vi "subFindProjects.vi"(8 "error in (no error)":errorcluster, 11 "SolutionBuilder in":refnum<class "SolutionBuilder.lvclass">) -> (0 "error out":errorcluster, 3 "SolutionBuilder out":refnum<class "SolutionBuilder.lvclass">)   [LabVIEW 2019, in "SolutionBuilder.lvlib" / "SolutionBuilder.lvclass"]
uses:
  SolutionBuilder.lvclass
  SolutionBuilder.lvclass/SolutionBuilder.ctl
  ProjectItem/ProjectItem.lvclass
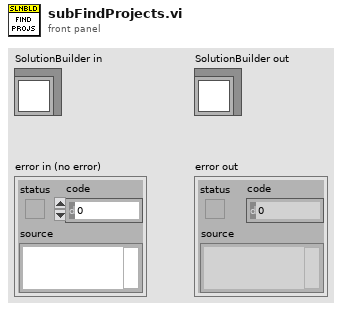
[diagram p1: front panel]
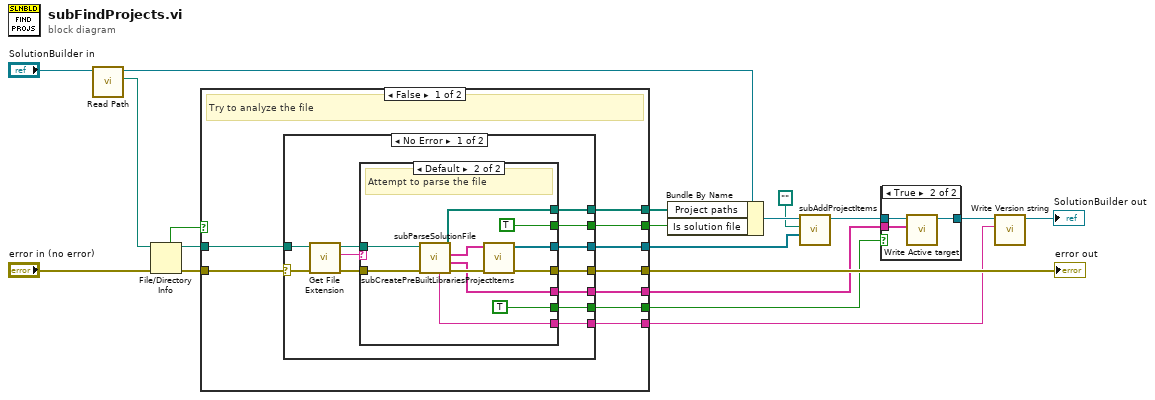
[diagram p0: block diagram]
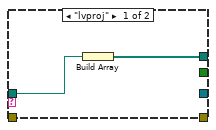
[diagram p3: hidden frame]
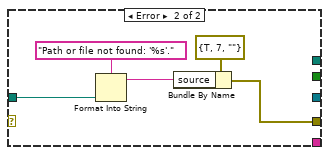
[diagram p4: hidden frame]
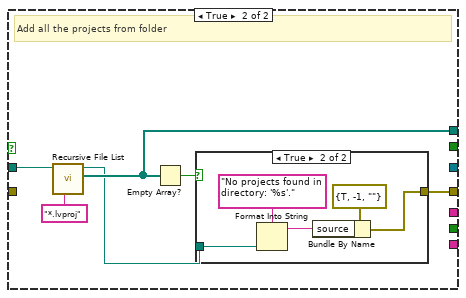
[diagram p5: hidden frame]
diagram:
  n1 = call "Read Path.vi"("SolutionBuilder in"="SolutionBuilder in") -> ("Path"=w15:path, "SolutionBuilder out"=w14:refnum<class "SolutionBuilder.lvclass">)  [unwired: 9 in]
  n2 = File/Directory Info(path=w15, error in="error in (no error)") -> (path out=w18:path, directory=w19:bool, error out=w17:errorcluster)  [unwired: 4 out]
  n3 = case shown="False" w19 {
    tunnel: [w26 w62] -> w11
    tunnel: w18 -> [w28 w61]
    tunnel: w17 -> [w27 _]
    tunnel: [w25 w63] -> w12
    tunnel: [w24 _] -> w8
    tunnel: [w23 _] -> w7
    tunnel: [w22 _] -> w5
    tunnel: [w21 _] -> w4
    tunnel: [w20 _] -> w1
    frame False {
      # "Try to analyze the file"
      n4 = case shown="No Error" w27 {
        selector: w27 -> [w39 _]
        tunnel: w28 -> [w38 w56]
        tunnel: [w40 _] -> w26
        tunnel: [w34 w55] -> w25
        tunnel: [w33 _] -> w24
        tunnel: [w32 _] -> w23
        tunnel: [w31 _] -> w22
        tunnel: [w30 _] -> w21
        tunnel: [w29 _] -> w20
        frame No Error {
          n5 = call <vilib>:"Get File Extension.vi"("error in (no error)"=w39, "file"=w38) -> ("error out"=w36:errorcluster, "lowercase file extension"=w35:string, "dup file"=w37:path)  [unwired: 5 in, 2 out]
          n6 = case shown="Default" w35 {
            tunnel: [w41 w53] -> w40
            tunnel: w37 -> [w42 w51]
            tunnel: w36 -> [_ w52]
            tunnel: [_ w48] -> w34
            tunnel: [_ w47] -> w33
            tunnel: [_ TRUE ("Is solution file")] -> w32
            tunnel: [_ w45] -> w31
            tunnel: [_ TRUE] -> w30
            tunnel: [_ w43] -> w29
            frame "lvproj" {
              n7 = Build Array(w42) -> (w41:path[])
            }
            frame Default {
              # "Attempt to parse the file"
              n8 = call "subParseSolutionFile.vi"("error in (no error)"=w52, "Solution file"=w51) -> ("error out"=w49:errorcluster, "Active targets"=w45:string[], "Lib definition strings"=w50:string[], "Projects"=w53:path[], "Version string"=w43:string)  [unwired: 5 in]
              n9 = call "subCreatePreBuiltLibrariesProjectItems.vi"("error in"=w49, "Lib definition strings"=w50) -> ("error out"=w48:errorcluster, "Pre-built libraries"=w47:refnum<class "ProjectItem.lvclass">[])  [unwired: 8 in]
            }
          }
        }
        frame Error {
          n10 = Format Into String(format string="Path or file not found: '%s'.", w56) -> (resulting string=w57:string)  [unwired: 2 in, 1 out]
          n11 = Bundle By Name(cluster=errorcluster {"status"=TRUE, "code"=7, "source"=""} ("t"), "source"=w57) -> (w55:errorcluster)
        }
      }
    }
    frame True {
      # "Add all the projects from folder"
      n12 = call <vilib>:"Recursive File List.vi"("pattern"="*.lvproj", "Folder Path"=w61) -> ("All Files in Dir"=w62:path[], "dup Folder Path"=w60:path)  [unwired: 5 in, 3 out]
      n13 = Empty Array?(array=w62) -> (empty?=w59:bool)
      n14 = case shown="True" w59 {
        tunnel: [_ w66] -> w63
        tunnel: w60 -> [_ w65]
        frame False {
        }
        frame True {
          n15 = Format Into String(format string="No projects found in directory: '%s'.", w65) -> (resulting string=w68:string)  [unwired: 2 in, 1 out]
          n16 = Bundle By Name(cluster=errorcluster {"status"=TRUE, "code"=-1, "source"=""} ("t"), "source"=w68) -> (w66:errorcluster)
        }
      }
    }
  }
  "error out" <- w12
  n17 = Bundle By Name(cluster=w14, "Project paths"=w11, "Is solution file"=w7) -> (w10:refnum<class "SolutionBuilder.lvclass">)
  n18 = call "subAddProjectItems.vi"("ProjectItems"=w8, "Owning project"=path "", "SolutionBuilder in"=w10) -> ("SolutionBuilder out"=w6:refnum<class "SolutionBuilder.lvclass">)  [unwired: 7 in, 1 out]
  n19 = case shown="True" w4 {
    tunnel: w6 -> [w70 w73]
    tunnel: [w70 w72] -> w3
    tunnel: w5 -> [_ w71]
    frame False {
    }
    frame True {
      n20 = call-dynamic "Write Active target.vi"("Active targets"=w71, "SolutionBuilder in"=w73) -> ("SolutionBuilder out"=w72:refnum<class "SolutionBuilder.lvclass">)  [unwired: 9 in]
    }
  }
  n21 = call "Write Version string.vi"("Version string"=w1, "SolutionBuilder in"=w3) -> ("SolutionBuilder out"=→"SolutionBuilder out":refnum<class "SolutionBuilder.lvclass">)  [unwired: 9 in]
